vi "Lookup Target Channels.vi"(6 "VolatusAPI":refnum<class "VolatusAPI.lvclass">, 8 "error in (no error)":errorcluster, 11 "LoggingControl in":refnum<class "GroupLoggingControl.lvclass">) -> (0 "error out":errorcluster, 3 "LoggingControl out":refnum<class "GroupLoggingControl.lvclass">)   [LabVIEW 2020, in "VolatusGUIElements.lvlib" / "GroupLoggingControl.lvclass"]
uses:
  GroupLoggingControl.lvclass
  Volatus/VolatusAPI/VolatusAPI.lvclass
  VolatusConfig/Meta Name.ctl
  GroupLoggingControl.lvclass/GroupLoggingControl.ctl
  Volatus/VolatusAPI/VolatusAPI.lvclass/VolatusAPI.ctl
  lv-vecto/Vecto/Group DBL/Group DBL.lvclass
  C:/dev/lv20CE/relink/lv-vecto/Vecto/Group/Group.lvclass
  VolatusConfig/VolatusConfigElement/VolatusConfigElement.lvclass/VolatusConfigElement.ctl
  VolatusConfig/VolatusConfigElement/Element.vi
  VolatusConfig/Node/Node Config.lvclass
  C:/dev/lv20CE/relink/lv-volatus/VolatusConfig/VolatusConfigElement/VolatusConfigElement.lvclass
  lv-cdm/CDM-Config/Config Element/Owner.vi
  lv-cdm/CDM-Config/Config Manager/Lookup Descendant.vi
  lv-cdm/CDM-Config/Config Filter/Config Lookup.lvclass
  VolatusConfig/Cluster/Cluster Config.lvclass
  VolatusConfig/VolatusConfigElement/VolatusConfigElement.lvclass
  VolatusConfig/Channel/Channel Config.lvclass
  VolatusConfig/VolatusConfig.lvlib
  lv-cdm/CDM-Config/Config Element/Config Element.lvclass
  C:/dev/lv20CE/relink/lv-volatus/VolatusConfig/Node/Node Config.lvclass
  C:/dev/lv20CE/relink/lv-vecto/Vecto/Group DBL/Group DBL.lvclass
  lv-vecto/Vecto/Channel DBL/Channel DBL.lvclass
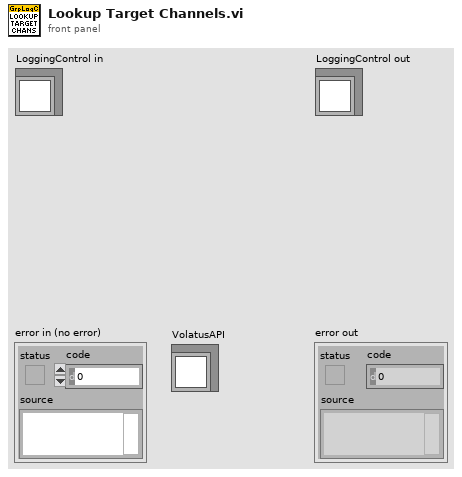
[diagram p1: front panel]
types:
  T1 = typedef "VolatusConfig.lvlib/Meta Name.ctl" = enum16{"VL_Type", "VL_Node_IP", "VL_Node_Type", "VL_Task_Type", "VL_Group_Type", "VL_Channel_Type", "VL_Channel_DataType", "VL_Config_Version", "VL_Overlay_Type", "VL_Config_Hash"}
  T2 = typedef "VolatusGUIElements.lvlib/GroupLoggingControl.lvclass/Status.ctl" = cluster{"Groups":T3[], "Targets":T6[]}
  T3 = typedef "VolatusGUIElements.lvlib/GroupLoggingControl.lvclass/Log Group.ctl" = cluster{"Status":T4, "Command Info":T5, "Logging":bool, "State":string}
  T4 = typedef "VolatusGUIElements.lvlib/GroupLoggingControl.lvclass/Log Group Status.ctl" = cluster{"Group":string, "Group Color":u32, "Button":bool}
  T5 = typedef "VolatusGUIElements.lvlib/GroupLoggingControl.lvclass/Command Info.ctl" = cluster{"Commanding":bool, "Cmd Time":dbl, "Group ID":string}
  T6 = typedef "VolatusGUIElements.lvlib/GroupLoggingControl.lvclass/Target Info.ctl" = cluster{"Node":string, "Node Color":u32, "Groups":T3[]}
  T7 = typedef "VectoConfig.lvlib/Channel Info.ctl" = cluster{"Name":string, "Group":string, "Owning Node":string, "Owning Task":string, "Resource":string}
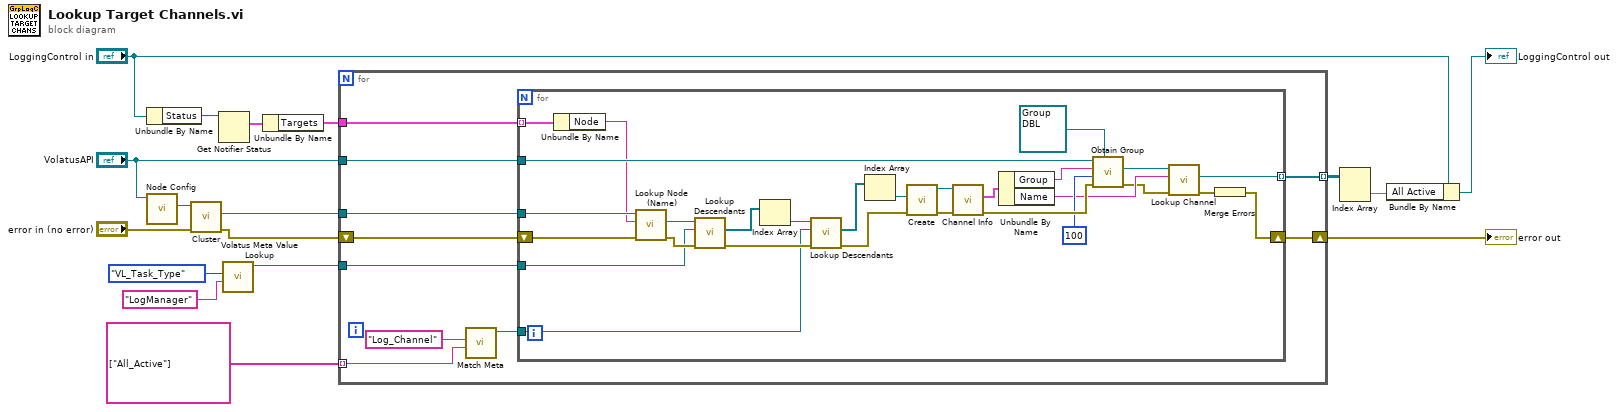
[diagram p0: block diagram]
diagram:
  n1 = Unbundle By Name("LoggingControl in") -> ("Status"=w2:refnum<notifier>)
  n2 = call "Node Config.vi"("VolatusAPI in"="VolatusAPI") -> ("Node Config"=w17:refnum<class "Node Config.lvclass">)  [unwired: 9 in, 1 out]
  n3 = call "Cluster.vi"("error in (no error)"="error in (no error)", "Node in"=w17) -> ("error out"=w14:errorcluster, "Cluster"=w16:refnum<class "Cluster Config.lvclass">)  [unwired: 7 in, 1 out]
  n4 = Get Notifier Status(notifier=w2) -> (current notification=w1:T2)  [unwired: 1 in, 4 out]
  n5 = call "Volatus Meta Value Lookup.vi"("Value"="LogManager", "Meta Name"=Meta_Name."VL_Task_Type") -> ("Config Lookup out"=w4:refnum<class "Config Lookup.lvclass">)  [unwired: 8 in, 1 out]
  n6 = Unbundle By Name(w1) -> ("Targets"=w15:T6[])
  n7 = for {
    tunnel: w16 -> [w27]
    tunnel: "VolatusAPI" -> [w24]
    tunnel: [w23] -> w9 mode=indexing
    shift-right: [w22] -> w7
    shift-left: w14 -> [w25]
    tunnel: string[] ["All_Active"] -> [w19] mode=indexing
    tunnel: w4 -> [w18]
    tunnel: w15 -> [w26]
    n8 = call "Match Meta.vi"("Value (Any)"=w19, "Name"="Log_Channel") -> ("Config Lookup out"=w20:refnum<class "Config Lookup.lvclass">)  [unwired: 8 in, 1 out]
    n9 = for {
      tunnel: w27 -> [w53]
      tunnel: w26 -> [w43] mode=indexing
      tunnel: w20 -> [w38]
      shift-right: [w34] -> w22
      shift-left: w25 -> [w52]
      tunnel: w24 -> [w48]
      tunnel: [w28] -> w23 mode=indexing
      tunnel: w18 -> [w40]
      n10 = Unbundle By Name(w43) -> ("Node"=w44:string)
      n11 = call "Lookup Node (Name).vi"("error in (no error)"=w52, "Node Name"=w44, "Cluster in"=w53) -> ("error out"=w41:errorcluster, "Node"=w42:refnum<class "Node Config.lvclass">)  [unwired: 6 in, 1 out]
      n12 = call "Lookup Descendants.vi"("error in (no error)"=w41, "Lookup"=w40, "VolatusConfigElement in"=w42) -> ("error out"=w55:errorcluster, "Descendants"=w39:refnum<class "Config Element.lvclass">[])  [unwired: 6 in, 1 out]
      n13 = Index Array(array=w39) -> (element=w35:refnum<class "Config Element.lvclass">)  [unwired: 1 in]
      n14 = call "Lookup Descendants.vi"("error in (no error)"=w55, "Lookup"=w38, "Config Element in"=w35) -> ("error out"=w36:errorcluster, "Descendants"=w37:refnum<class "Config Element.lvclass">[])  [unwired: 6 in, 1 out]
      n15 = Index Array(array=w37) -> (element=w51:refnum<class "Config Element.lvclass">)  [unwired: 1 in]
      n16 = call "Create.vi"("error in (no error)"=w36, "Element"=w51) -> ("error out"=w49:errorcluster, "Channel out"=w50:refnum<class "Channel Config.lvclass">)  [unwired: 8 in]
      n17 = call "Channel Info.vi"("error in (no error)"=w49, "Channel in"=w50) -> ("error out"=w54:errorcluster, "Channel Info"=w47:T7)  [unwired: 7 in, 1 out]
      n18 = Unbundle By Name(w47) -> ("Group"=w45:string, "Name"=w31:string)
      n19 = call "Obtain Group.vi"("Group Type (Abstract)"=refnum<class "Group DBL.lvclass"> refnum ("Vecto.lvlib:StringGroup.lvclass"), "error in (no error)"=w54, "Timeout ms (5000)"=u32 100, "Group Name"=w45, "VolatusAPI in"=w48) -> ("error out"=w30:errorcluster, "Group"=w32:refnum<class "Group DBL.lvclass">)  [unwired: 4 in, 1 out]
      n20 = call "Lookup Channel.vi"("error in (no error)"=w30, "Channel Name"=w31, "Group in"=w32) -> ("error out"=w29:errorcluster, "Channel"=w28:refnum<class "Channel DBL.lvclass">)  [unwired: 6 in, 1 out]
      n21 = Merge Errors(w29) -> (w34:errorcluster)
    }
  }
  "error out" <- w7
  n22 = Index Array(array=w9) -> (element=w8:refnum<class "Channel DBL.lvclass">[])  [unwired: 2 in]
  n23 = Bundle By Name(cluster="LoggingControl in", "All Active"=w8) -> (→"LoggingControl out":refnum<class "GroupLoggingControl.lvclass">)
